vi "Get Status Error Channel Data References.vi"(8 "error in":errorcluster, 11 "custom device ref in":T1 format="%.0x") -> (0 "error out":errorcluster, 2 "status channel data references":T1[](array[typedef]) format="%.0x", 3 "custom device ref out":T1 format="%.0x")   [LabVIEW 2020]
uses:
  <vilib>/NI VeriStand/Custom Device API/Custom Device Item Ref.ctl
  Scripting/Ballard/Ballard ARINC 429 Scripting.lvlib
  <vilib>/NI VeriStand/Custom Device API/Custom Device API.lvlib
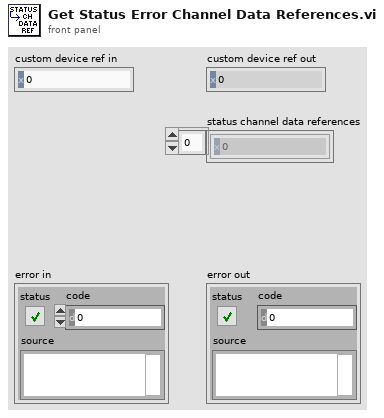
[diagram p1: front panel]
types:
  T1 = typedef "Custom Device API.lvlib/Custom Device Item Ref.ctl" = u64
  T2 = cluster{"gap":T1, "parity":T1, "long word":T1, "bit timing":T1, "timeout":T1}
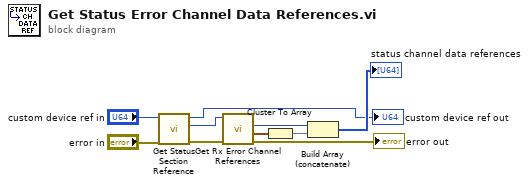
[diagram p0: block diagram]
diagram:
  n1 = call "Get Status Section Reference.vi"("error in"="error in", "Ballard ARINC 429 ref"="custom device ref in") -> ("error out"=w8:errorcluster, "status section reference"=w9:T1, "Ballard ARINC 429 ref out"=→"custom device ref out":T1)  [unwired: 7 in]
  n2 = call "Get Rx Error Channel References.vi"("error in"=w8, "status reference in"=w9) -> ("error out"=→"error out":errorcluster, "Rx specific error count references"=w6:T2, "Rx error count reference"=w4:T1)  [unwired: 6 in, 1 out]
  n3 = Cluster To Array(cluster=w6) -> (array=w5:T1[])
  n4 = Build Array (concatenate)(w4, w5) -> (→"status channel data references":T1[])
